vi "getMissingCellPolicy.vi"(8 "error in (no error)":errorcluster) -> (0 "error out":errorcluster, 3 "CREATE_NULL_AS_BLANK":refnum<k24>)   [LabVIEW 2017, in "LabVIEW NPOI.lvlib" / "MS-Excel.lvclass"]
uses:
  MS-Excel.lvclass
  C:/Program Files (x86)/National Instruments/LabVIEW 2017/vi.lib/BenjaminR/LabVIEW NPOI/lib/NPOI 2.1.1/NPOI.dll
  Program Files (x86)/National Instruments/LabVIEW 2017/vi.lib/BenjaminR/LabVIEW NPOI/lib/NPOI 2.1.1/NPOI.dll
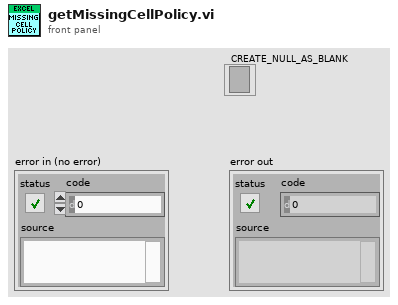
[diagram p1: front panel]
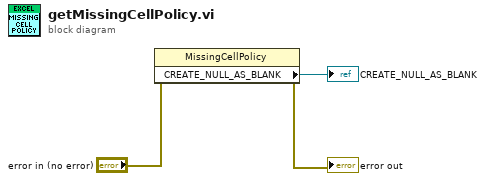
[diagram p0: block diagram]
diagram:
  n1 = property class="MissingCellPolicy"(error in="error in (no error)") -> (error out=→"error out":errorcluster, "CREATE_NULL_AS_BLANK"=→"CREATE_NULL_AS_BLANK":refnum<k24>)  [unwired: 1 in, 1 out]
